vi "Module Init.vi"(8 "error in (no error)":errorcluster, 11 "Historian Module in":refnum<class "Historian Module.lvclass">) -> (0 "error out":errorcluster, 3 "Historian Module out":refnum<class "Historian Module.lvclass">)   [LabVIEW 2020, in "VolatusHistorian.lvlib" / "Historian Module.lvclass"]
uses:
  Historian Module.lvclass
  Volatus/Module/Module.lvclass
  C:/dev/lv20CE/relink/lv-volatus/Volatus/Module/Module.lvclass
  History Data Controller/History Data Controller.lvclass
  Volatus/VolatusAPI/VolatusAPI.lvclass
  C:/dev/lv20CE/relink/lv-http-server/HTTP Server/Handler/Handler.lvclass
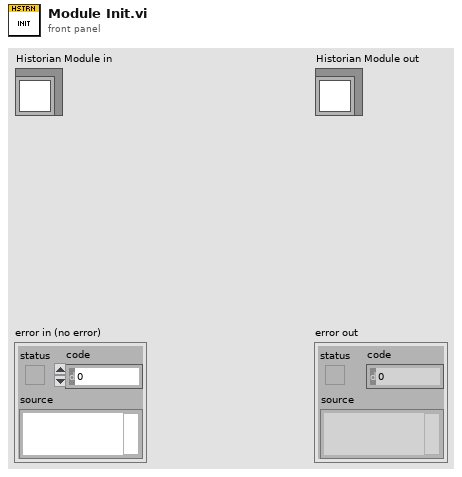
[diagram p1: front panel]
types:
  T1 = typedef "VolatusHistorian.lvlib/Historian Module.lvclass/Historian Role.ctl" = enum16{"Primary", "Local"}
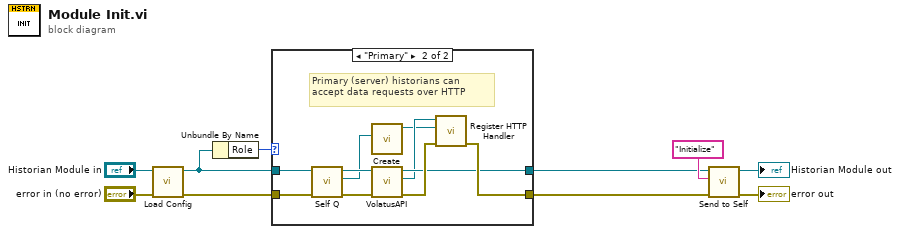
[diagram p0: block diagram]
diagram:
  n1 = call "Load Config.vi"("error in (no error)"="error in (no error)", "Historian Module in"="Historian Module in") -> ("error out"=w9:errorcluster, "Historian Module out"=w2:refnum<class "Historian Module.lvclass">)  [unwired: 8 in]
  n2 = Unbundle By Name(w2) -> ("Role"=w1:T1)
  n3 = case shown="\"Primary\"" w1 {
    tunnel: [w11 w20] -> w10
    tunnel: w9 -> [w11 w19]
    tunnel: [w12 w16] -> w3
    tunnel: w2 -> [w12 w13]
    frame "Local" {
      # "Local historians don't accept remote requests over HTTP"
    }
    frame "Primary" {
      # "Primary (server) historians can accept data requests over HTTP"
      n4 = call "Self Q.vi"("Module in"=w13) -> ("Self Q"=w17:refnum<class "MessageQ.lvclass">, "Module out"=w18:refnum<class "Historian Module.lvclass">)  [unwired: 9 in]
      n5 = call "Create.vi"("Historian MsgQ"=w17) -> ("History Data Controller out"=w14:refnum<class "History Data Controller.lvclass">)  [unwired: 9 in, 1 out]
      n6 = call "VolatusAPI.vi"("Module in"=w18) -> ("VolatusAPI"=w15:refnum<class "VolatusAPI.lvclass">, "Module out"=w16:refnum<class "Historian Module.lvclass">)  [unwired: 9 in]
      n7 = call "Register HTTP Handler.vi"("error in (no error)"=w19, "Handler"=w14, "VolatusAPI in"=w15) -> ("error out"=w20:errorcluster)  [unwired: 7 in, 1 out]
    }
  }
  n8 = call "Send to Self.vi"("error in (no error)"=w10, "Message ID"="Initialize", "Module in"=w3) -> ("error out"=→"error out":errorcluster, "Module out"=→"Historian Module out":refnum<class "Historian Module.lvclass">)  [unwired: 7 in]
